vi "lvmcp_casenames.vi"() -> ()   [LabVIEW 2015]
panel:
  out "error out":errorcluster
  out "names":string[](array[string])
  in  "reference":refnum<vi>
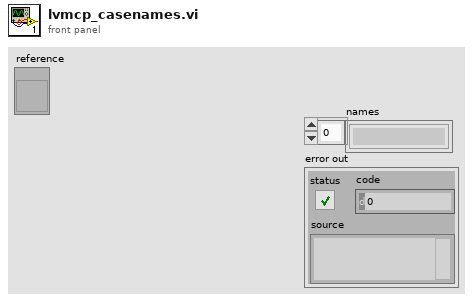
[diagram p1: front panel]
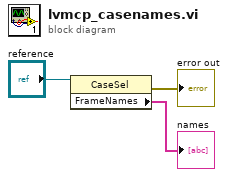
[diagram p0: block diagram]
diagram:
  n1 = property class="CaseSel"(reference="reference") -> (error out=→"error out":errorcluster, "FrameNames"=→"names":string[])  [unwired: 1 in, 1 out]
